vi "set HO BandWidth.vi"(8 "error in (no error)":errorcluster caption="에러 입력(에러 없음)", 9 "LTE Channel Type":T2, 10 "BandWidth":T1, 11 "LTE 입력":refnum<class "LTE.lvclass">) -> (0 "error out":errorcluster caption="에러 출력", 3 "LTE 출력":refnum<class "LTE.lvclass">)   [LabVIEW 2023, in "ANRITSU Call Box.lvlib" / "LTE.lvclass"]
uses:
  LTE.lvclass
  LTE.lvclass/LTE.ctl
  Type Definition/LTE Channel Type.ctl
  ANRITSU Call Box.lvlib
  Type Definition/LTE Supported BandWidth.ctl
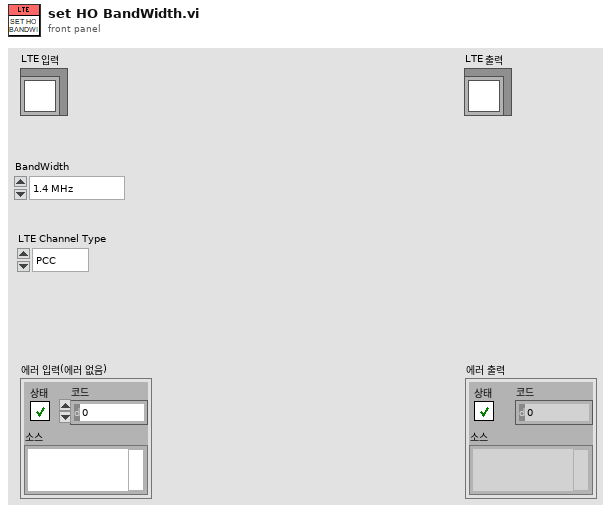
[diagram p1: front panel]
types:
  T1 = typedef "ANRITSU Call Box.lvlib/LTE Supported BandWidth.ctl" = enum16{"1.4 MHz", "3 MHz", "5 MHz", "10 MHz", "15 MHz", "20 MHz"}
  T2 = typedef "ANRITSU Call Box.lvlib/LTE Channel Type.ctl" = enum16{"PCC", "SCC1", "SCC2", "SCC3"}
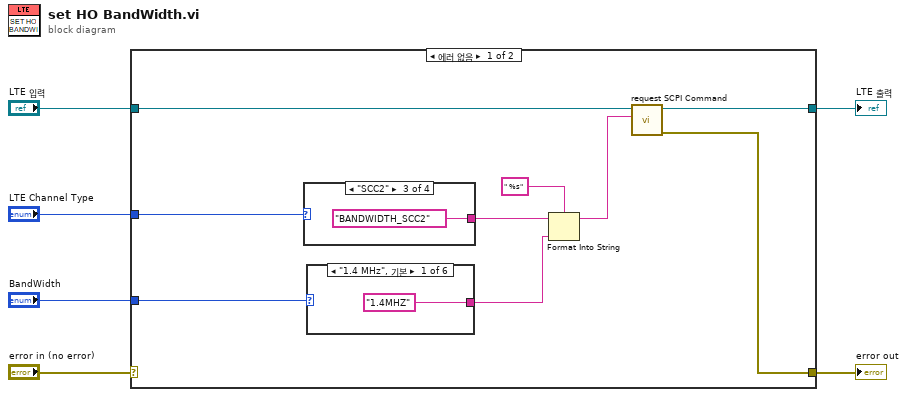
[diagram p0: block diagram]
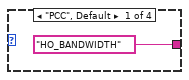
[diagram p2: hidden frame]
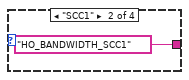
[diagram p3: hidden frame]
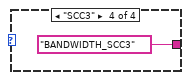
[diagram p4: hidden frame]
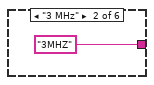
[diagram p5: hidden frame]
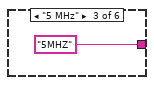
[diagram p6: hidden frame]
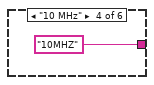
[diagram p7: hidden frame]
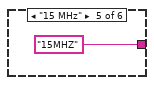
[diagram p8: hidden frame]
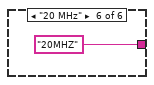
[diagram p9: hidden frame]
diagram:
  n1 = case shown="에러 없음" "error in (no error)" {
    selector: "error in (no error)" -> [_ w27]
    tunnel: [w9 w27] -> w5
    tunnel: [w10 w26] -> w3
    tunnel: "LTE 입력" -> [w11 w26]
    tunnel: "BandWidth" -> [w8 _]
    tunnel: "LTE Channel Type" -> [w7 _]
    frame No Error {
      n2 = case shown="\"SCC2\"" w7 {
        tunnel: ["HO_BANDWIDTH" ("string") "HO_BANDWIDTH_SCC1" ("string") "BANDWIDTH_SCC2" ("string") "BANDWIDTH_SCC3" ("string")] -> w15
        frame "PCC", Default {
        }
        frame "SCC1" {
        }
        frame "SCC2" {
        }
        frame "SCC3" {
        }
      }
      n3 = case shown="\"1.4 MHz\", 기본" w8 {
        tunnel: ["1.4MHZ" "3MHZ" "5MHZ" "10MHZ" "15MHZ" "20MHZ"] -> w13
        frame "1.4 MHz", Default {
        }
        frame "3 MHz" {
        }
        frame "5 MHz" {
        }
        frame "10 MHz" {
        }
        frame "15 MHz" {
        }
        frame "20 MHz" {
        }
      }
      n4 = Format Into String(format string=" %s", initial string=w15, w13) -> (resulting string=w12:string)  [unwired: 1 in, 1 out]
      n5 = call "request SCPI Command.vi"("SCPI Command"=w12, "LTE in"=w11) -> ("error out"=w9:errorcluster, "LTE out"=w10:refnum<class "LTE.lvclass">)  [unwired: 8 in]
    }
    frame Error {
    }
  }
  "error out" <- w5
  "LTE 출력" <- w3
